vi "To XML.vi"(8 "error in (no error)":errorcluster, 11 "Serializable in":refnum<class "Serializable.lvclass">) -> (0 "error out":errorcluster, 2 "XML":string)   [LabVIEW 2013, in "JUnit XML.lvlib" / "Serializable.lvclass"]
doc: "Serializes a JUnit object to XML."
uses:
  Serializable.lvclass
  <vilib>/xml/NI_XML.lvlib
  <resource>/objmgr/DOMUserDefRef.rc
  <vilib>/xml/Close Reference(Node).vi
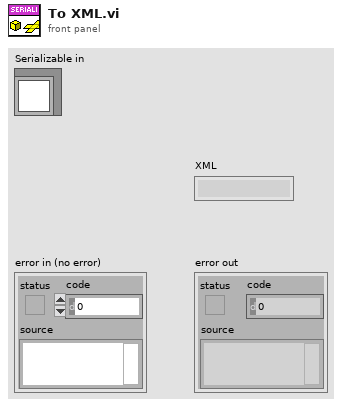
[diagram p1: front panel]
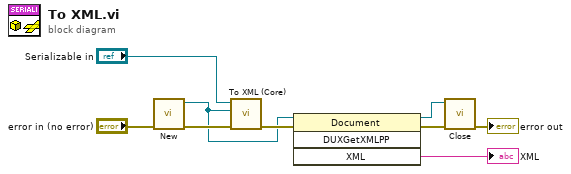
[diagram p0: block diagram]
diagram:
  n1 = call <vilib>:"New.vi"("error in (no error)"="error in (no error)") -> ("error out"=w8:errorcluster, "DOM document out"=w4:refnum<k20>)  [unwired: 7 in]
  n2 = call-dynamic "To XML (Core).vi"("error in (no error)"=w8, "Parent"=w4, "Serializable in"="Serializable in") -> ("error out"=w6:errorcluster)  [unwired: 8 in]
  n3 = invoke class="Document" method="DUXGetXMLPP"(reference=w4, error in=w6) -> (reference out=w1:refnum<k20>, error out=w5:errorcluster, "XML"=→"XML":string)  [unwired: 2 in, 1 out]
  n4 = call-poly <vilib>:"Close.vi"("error in (no error)"=w5, "node"=w1) -> ("error out"=→"error out":errorcluster)  [unwired: 7 in]
